vi "Generic DAQmx DIO Shutter Engine.vi"(0 "Unique Notifier Name":string="Not a Name", 11 "DIO Lines":string[](array[string])) -> ()   [LabVIEW 2016]
uses:
  Shutter Controls/Shutter Notifier Element.ctl
  Shutter Controls/Shutter Actions.ctl
  <vilib>/DAQmx/write.llb/DAQmx Write (Digital Bool 1Line 1Point).vi
  <vilib>/DAQmx/read.llb/DAQmx Read (Digital Bool 1Line 1Point).vi
  <vilib>/DAQmx/create/channels.llb/DAQmx Create Channel (DO-Digital Output).vi
  <vilib>/DAQmx/miscellaneous.llb/DAQmx Fill In Error Info.vi
  <vilib>/DAQmx/create/channels.llb/DAQmx Create Channel (DI-Digital Input).vi
panel:
  in  "Quit":bool
  in  "Shutter":bool
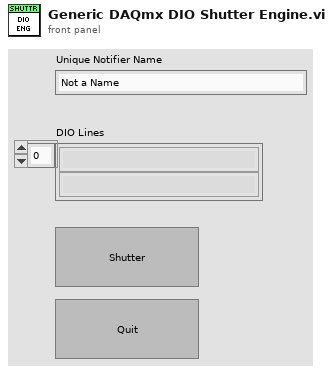
[diagram p1: front panel]
types:
  T1 = typedef "Shutter Notifier Element.ctl" = cluster{"Action":T2, "Status":T2, "Received?":bool}
  T2 = typedef "Shutter Actions.ctl" = enum16{"Open", "Close", "Toggle", "Status", "Quit"}
  T3 = enum32{"Invalid", "Standard", "Closed", "Hidden", "Minimized", "Maximized"}
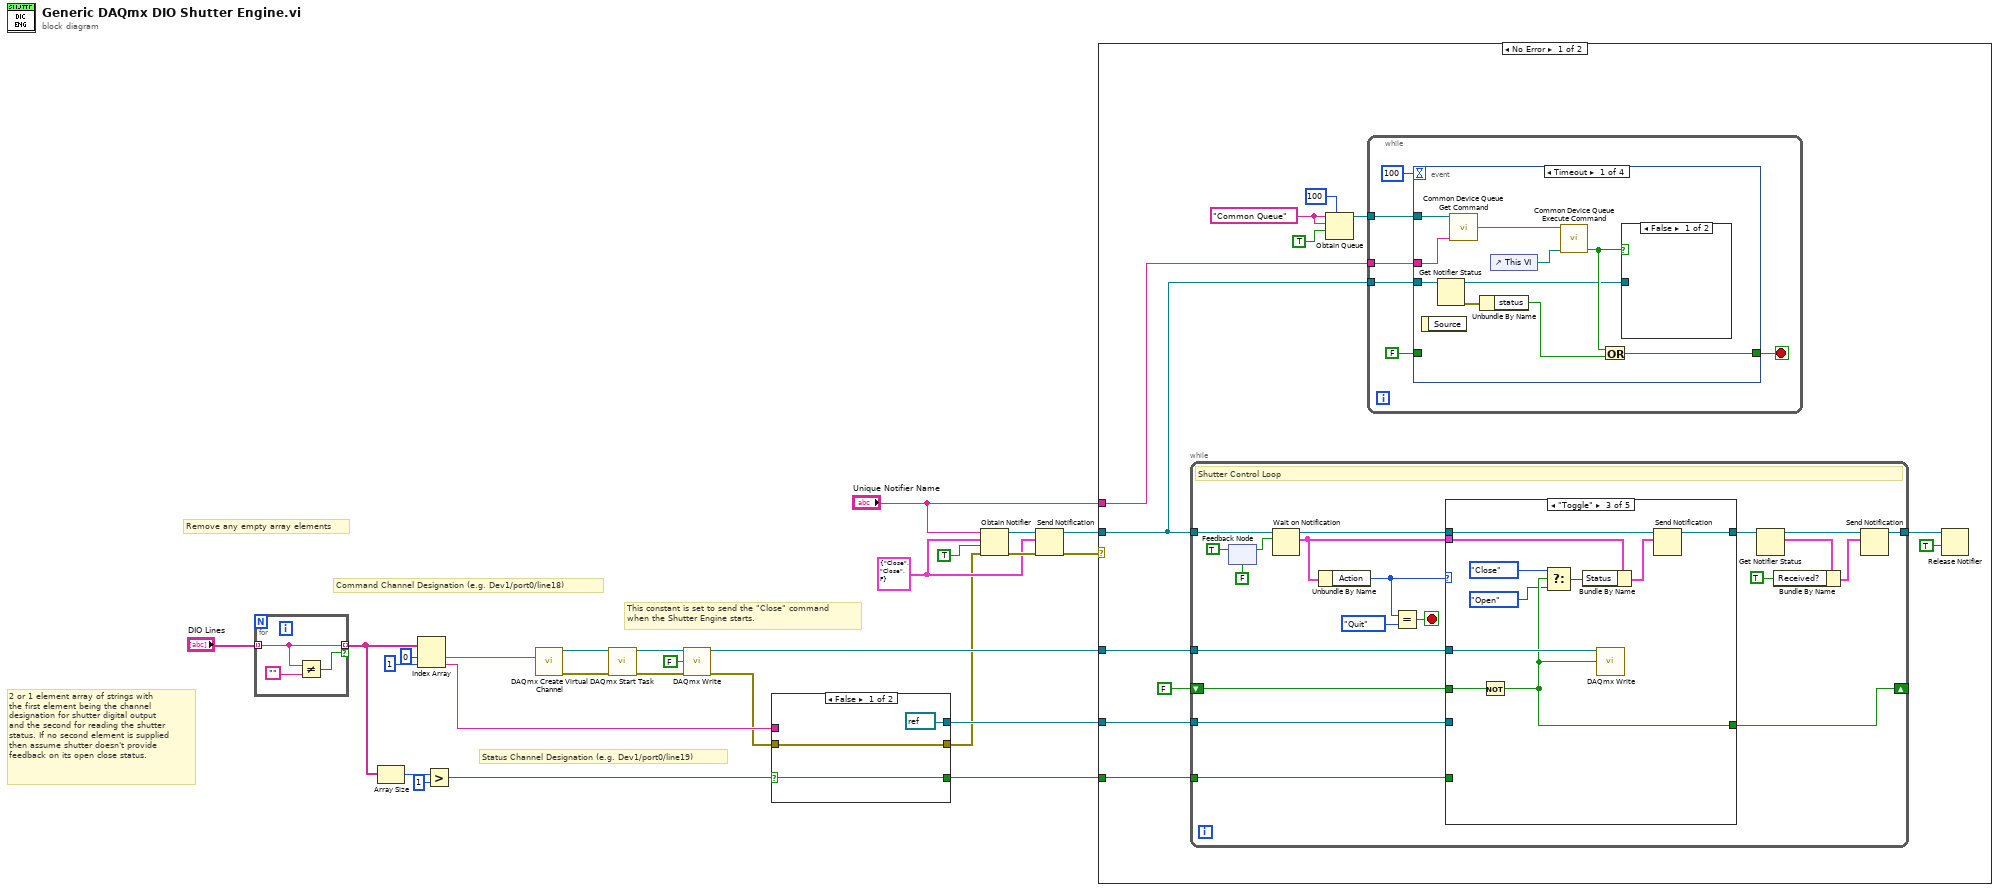
[diagram p0: block diagram]
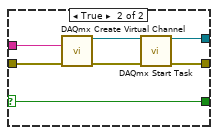
[diagram p2: hidden frame]
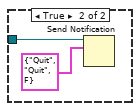
[diagram p3: hidden frame]
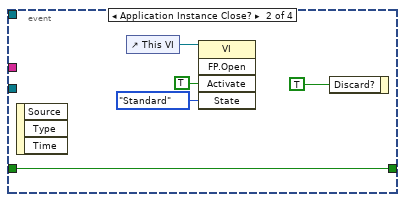
[diagram p4: hidden frame]
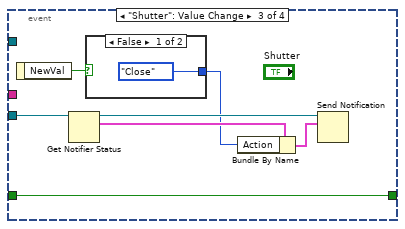
[diagram p5: hidden frame]
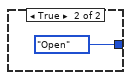
[diagram p6: hidden frame]
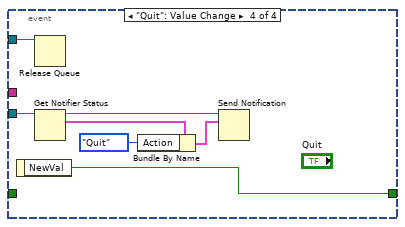
[diagram p7: hidden frame]
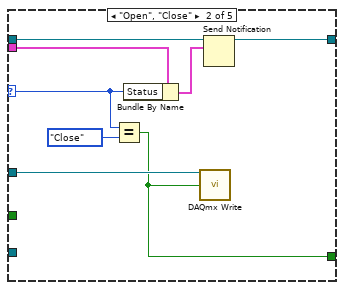
[diagram p9: hidden frame]
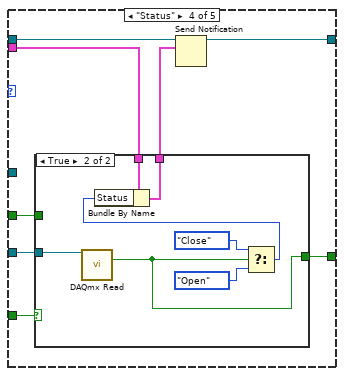
[diagram p10: hidden frame]
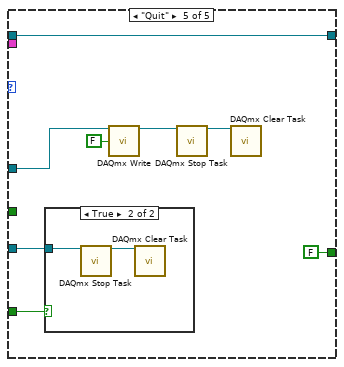
[diagram p12: hidden frame]
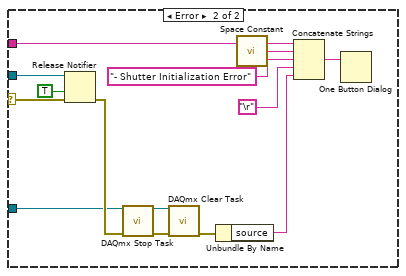
[diagram p14: hidden frame]
diagram:
  w16 = T1 {"Action"=enum."Close", "Status"=enum."Close", "Received?"=FALSE} ("Shutter Notifier Element")
  # "Remove any empty array elements"
  # "This constant is set to send the \"Close\" command\nwhen the Shutter Engine starts."
  # "2 or 1 element array of strings with\nthe first element being the channel\ndesignation for shutter digital output\nand the second for reading the shutter\nstatus. If no second element is supplied\nthen assume shutter doesn't provide\nfeedback on its open close status."
  # "Status Channel Designation (e.g. Dev1/port0/line19)"
  # "Command Channel Designation (e.g. Dev1/port0/line18)"
  n1 = for {
    tunnel: "DIO Lines" -> [w28] mode=indexing
    tunnel: [w28] -> w1 mode=indexing if=w27
    n2 = Not Equal?(x=w28, y="") -> (x != y?=w27:bool)
  }
  n3 = Array Size(array=w1) -> (size(s)=w9:i32)
  n4 = Index Array(array=w1, index #1=0 ("index"), index #2=1 ("index")) -> (element #1=w4:string, element #2=w10:string)
  n5 = Greater?(x=w9, y=1) -> (0:w3:bool)
  n6 = call-poly <vilib>:"DAQmx Create Virtual Channel.vi"("lines"=w4) -> ("task out"=w25:refnum<k21>, "error out"=w26:errorcluster)  [unwired: 4 in, 9 out]
  n7 = call <vilib>:"DAQmx Start Task.vi"("task/channels in"=w25, "error in"=w26) -> ("task out"=w20:refnum<k21>, "error out"=w21:errorcluster)  [unwired: 12 out]
  n8 = call-poly <vilib>:"DAQmx Write.vi"("task/channels in"=w20, "data"=FALSE, "error in"=w21) -> ("task out"=w18:refnum<k21>, "error out"=w7:errorcluster)  [unwired: 1 in, 10 out]
  n9 = case shown="False" w3 {
    selector: w3 -> [w30 w33]
    tunnel: [refnum<k21> refnum ("task out") w37] -> w15
    tunnel: w10 -> [_ w36]
    tunnel: w7 -> [w31 w35]
    tunnel: [w31 w34] -> w6
    tunnel: [w30 w33] -> w5
    frame False {
    }
    frame True {
      n10 = call-poly <vilib>:"DAQmx Create Virtual Channel.vi"("lines"=w36, "error in"=w35) -> ("task out"=w39:refnum<k21>, "error out"=w38:errorcluster)  [unwired: 3 in, 9 out]
      n11 = call <vilib>:"DAQmx Start Task.vi"("task/channels in"=w39, "error in"=w38) -> ("task out"=w37:refnum<k21>, "error out"=w34:errorcluster)  [unwired: 12 out]
    }
  }
  n12 = Obtain Notifier(name (unnamed)="Unique Notifier Name", notification data type=w16, create if not found? (T)=TRUE, error in (no error)=w6) -> (notifier out=w23:refnum<notifier>, error out=w22:errorcluster)  [unwired: 1 out]
  n13 = Send Notification(notification=w16, notifier=w23, error in (no error)=w22) -> (notifier out=w17:refnum<notifier>, error out=w14:errorcluster)
  n14 = case shown="No Error" w14 {
    selector: w14 -> [_ w164]
    tunnel: w18 -> [w51 w166]
    tunnel: w17 -> [w46 w167]
    tunnel: w15 -> [w48 _]
    tunnel: "Unique Notifier Name" -> [w45 w163]
    tunnel: w5 -> [w47 _]
    frame No Error {
      w43 = "Common Queue" ("Unique Notifier Name")
      n15 = while {
        tunnel: w46 -> [w100]
        tunnel: w51 -> [w108]
        tunnel: [w102] -> w49
        tunnel: w48 -> [w101]
        tunnel: w47 -> [w93]
        shift-right: [w91] -> _
        shift-left: FALSE -> [w92]
        stop <- w109 stop-if-true
        # "Shutter Control Loop"
        n16 = feedback #1(FALSE) -> (w96:bool)
        n17 = feedback-in #1(TRUE) -> ()
        n18 = Wait on Notification(notifier=w100, ignore previous (F)=w96) -> (notifier out=w99:refnum<notifier>, notification=w95:T1)  [unwired: 2 in, 2 out]
        n19 = Unbundle By Name(w95) -> ("Action"=w94:T2)
        n20 = Equal?(x=w94, y=Shutter_Actions."Quit") -> (x = y?=w109:bool)
        n21 = case shown="\"Toggle\"" w94 {
          selector: w94 -> [_ w114 _ _ _]
          tunnel: w99 -> [w112 w117 w127 w134 w155]
          tunnel: w108 -> [_ w118 w130 _ w153]
          tunnel: [w112 w119 w126 w136 w155] -> w105
          tunnel: w101 -> [_ _ _ w138 w150]
          tunnel: w95 -> [_ w116 w125 w135 _]
          tunnel: w93 -> [_ _ _ w133 w149]
          tunnel: w92 -> [w111 _ w129 w132 _]
          tunnel: [w111 w113 w124 w131 FALSE ("data")] -> w91
          frame Default {
          }
          frame "Open", "Close" {
            n22 = Equal?(x=w114, y=Shutter_Actions."Close") -> (x = y?=w113:bool)
            n23 = Bundle By Name(cluster=w116, "Status"=w114) -> (w120:T1)
            n24 = call-poly <vilib>:"DAQmx Write.vi"("task/channels in"=w118, "data"=w113) -> ()  [unwired: 2 in, 12 out]
            n25 = Send Notification(notification=w120, notifier=w117) -> (notifier out=w119:refnum<notifier>)  [unwired: 1 in, 1 out]
          }
          frame "Toggle" {
            n26 = Not(x=w129) -> (.not. x?=w124:bool)
            n27 = Select(t=Shutter_Actions."Close" ("Status"), s=w124, f=Shutter_Actions."Open" ("Status")) -> (s? t:f=w121:T2)
            n28 = Bundle By Name(cluster=w125, "Status"=w121) -> (w128:T1)
            n29 = call-poly <vilib>:"DAQmx Write.vi"("task/channels in"=w130, "data"=w124) -> ()  [unwired: 2 in, 12 out]
            n30 = Send Notification(notification=w128, notifier=w127) -> (notifier out=w126:refnum<notifier>)  [unwired: 1 in, 1 out]
          }
          frame "Status" {
            n31 = case shown="True" w133 {
              tunnel: w138 -> [_ w147]
              tunnel: [w140 w144] -> w137
              tunnel: w135 -> [w140 w142]
              tunnel: w132 -> [w139 _]
              tunnel: [w139 w141] -> w131
              frame False {
              }
              frame True {
                n32 = call-poly <vilib>:"DAQmx Read.vi"("task/channels in"=w147) -> ("data"=w141:bool)  [unwired: 12 in, 2 out]
                n33 = Select(t=Shutter_Actions."Close" ("Shutter Status"), s=w141, f=Shutter_Actions."Open" ("Shutter Status")) -> (s? t:f=w143:T2)
                n34 = Bundle By Name(cluster=w142, "Status"=w143) -> (w144:T1)
              }
            }
            n35 = Send Notification(notification=w137, notifier=w134) -> (notifier out=w136:refnum<notifier>)  [unwired: 1 in, 1 out]
          }
          frame "Quit" {
            n36 = case shown="True" w149 {
              tunnel: w150 -> [_ w157]
              frame False {
              }
              frame True {
                n37 = call <vilib>:"DAQmx Stop Task.vi"("task/channels in"=w157) -> ("task out"=w156:refnum<k21>)  [unwired: 13 in, 1 out]
                n38 = call <vilib>:"DAQmx Clear Task.vi"("task in"=w156) -> ()  [unwired: 1 in, 14 out]
              }
            }
            n39 = call-poly <vilib>:"DAQmx Write.vi"("task/channels in"=w153, "data"=FALSE) -> ("task out"=w151:refnum<k21>)  [unwired: 2 in, 11 out]
            n40 = call <vilib>:"DAQmx Stop Task.vi"("task/channels in"=w151) -> ("task out"=w152:refnum<k21>)  [unwired: 13 in, 1 out]
            n41 = call <vilib>:"DAQmx Clear Task.vi"("task in"=w152) -> ()  [unwired: 1 in, 14 out]
          }
        }
        n42 = Get Notifier Status(notifier=w105) -> (notifier out=w103:refnum<notifier>, current notification=w106:T1)  [unwired: 1 in, 3 out]
        n43 = Bundle By Name(cluster=w106, "Received?"=TRUE) -> (w107:T1)
        n44 = Send Notification(notification=w107, notifier=w103) -> (notifier out=w102:refnum<notifier>)  [unwired: 1 in, 1 out]
      }
      n45 = Obtain Queue(max queue size (-1, unlimited)=100, name (unnamed)=w43, element data type=w43, create if not found? (T)=TRUE) -> (queue out=w40:refnum<queue>)  [unwired: 1 in, 2 out]
      n46 = while {
        tunnel: w40 -> [w57]
        tunnel: w46 -> [w54]
        tunnel: w45 -> [w52]
        stop <- w53 stop-if-true
        n47 = event shown="[0] Timeout" {
          selector: _ -> [_ _ _ _]
          dyn-events: _ -> [_ _ _ _]
          timeout: 100 -> [_ _ _ _]
          tunnel: w57 -> [w65 _ _ w84]
          tunnel: FALSE -> [_ w74 w77 _]
          tunnel: w54 -> [w67 _ w81 w85]
          tunnel: [w60 w74 w77 w90] -> w53
          tunnel: w52 -> [w64 _ _ _]
          event Timeout {
            n48 = event-data() -> ()  [unwired: 1 in, 1 out]
            n49 = Get Notifier Status(notifier=w67) -> (notifier out=w58:refnum<notifier>, error out=w66:errorcluster)  [unwired: 1 in, 3 out]
            n50 = call "Common Device Queue Get Command.vi"("Common Queue"=w65, "Notifier Name"=w64) -> ("Command"=w63:string)  [unwired: 12 in, 1 out]
            n51 = Unbundle By Name(w66) -> ("status"=w61:bool)
            n52 = control-ref of="This VI"() -> (w62:refnum<vi>)
            n53 = call "Common Device Queue Execute Command.vi"("Common Command"=w63, "VI Refnum"=w62) -> ("Quit?"=w59:bool)  [unwired: 12 in, 1 out]
            n54 = Or(x=w59, y=w61) -> (x .or. y?=w60:bool)
            n55 = case shown="False" w59 {
              tunnel: w58 -> [_ w69]
              frame False {
              }
              frame True {
                n56 = Send Notification(notification=T1 {"Action"=enum."Quit", "Status"=enum."Quit", "Received?"=FALSE} ("Shutter Notifier Element"), notifier=w69) -> ()  [unwired: 1 in, 2 out]
              }
            }
          }
          event Application Instance Close? {
            n57 = event-data() -> ()  [unwired: 1 in, 3 out]
            n58 = control-ref of="This VI"() -> (w71:refnum<vi>)
            n59 = invoke class="VI" method="FP.Open"(reference=w71, "Activate"=TRUE ("Activate?"), "State"=T3."Standard") -> ()  [unwired: 2 in, 5 out]
            n60 = event-data("Discard?"=TRUE) -> ()  [unwired: 1 in, 1 out]
          }
          event "Shutter": Value Change {
            n61 = event-data() -> ("NewVal"=w76:bool)  [unwired: 1 in]
            n62 = Get Notifier Status(notifier=w81) -> (notifier out=w80:refnum<notifier>, current notification=w79:T1)  [unwired: 1 in, 3 out]
            n63 = case shown="False" w76 {
              tunnel: [Shutter_Actions."Close" ("Action") Shutter_Actions."Open" ("Action")] -> w75
              frame False {
              }
              frame True {
              }
            }
            n64 = Bundle By Name(cluster=w79, "Action"=w75) -> (w78:T1)
            n65 = Send Notification(notification=w78, notifier=w80) -> ()  [unwired: 1 in, 2 out]
          }
          event "Quit": Value Change {
            n66 = event-data() -> ("NewVal"=w90:bool)  [unwired: 1 in]
            n67 = Release Queue(queue=w84) -> ()  [unwired: 2 in, 3 out]
            n68 = Get Notifier Status(notifier=w85) -> (notifier out=w89:refnum<notifier>, current notification=w88:T1)  [unwired: 1 in, 3 out]
            n69 = Bundle By Name(cluster=w88, "Action"=Shutter_Actions."Quit") -> (w87:T1)
            n70 = Send Notification(notification=w87, notifier=w89) -> ()  [unwired: 1 in, 2 out]
          }
        }
      }
      n71 = Release Notifier(notifier=w49, force destroy? (F)=TRUE) -> ()  [unwired: 1 in, 3 out]
    }
    frame Error {
      n72 = Release Notifier(notifier=w167, force destroy? (F)=TRUE, error in (no error)=w164) -> (error out=w168:errorcluster)  [unwired: 2 out]
      n73 = call <vilib>:"DAQmx Stop Task.vi"("task/channels in"=w166, "error in"=w168) -> ("task out"=w170:refnum<k21>, "error out"=w169:errorcluster)  [unwired: 12 in]
      n74 = call <vilib>:"DAQmx Clear Task.vi"("task in"=w170, "error in"=w169) -> ("error out"=w165:errorcluster)  [unwired: 13 out]
      n75 = Unbundle By Name(w165) -> ("source"=w158:string)
      n76 = call <vilib>:"Space Constant.vi"() -> ("String"=w161:string)
      n77 = Concatenate Strings(w163, w161, "- Shutter Initialization Error" ("string"), "\r", w158) -> (w162:string)
      n78 = One Button Dialog(message=w162) -> ()  [unwired: 1 in, 1 out]
    }
  }
